vi "Serialize Proto.vi"(0 "protoFile ref in":u64, 3 "error in (no error)":errorcluster) -> (7 "protoFile ref out":u64, 8 "outBuffer":string, 10 "error out":errorcluster)   [LabVIEW 2019, in "gRPC Template Creation Utility.lvlib"]
uses:
  gRPC Template Creation Utility.lvlib
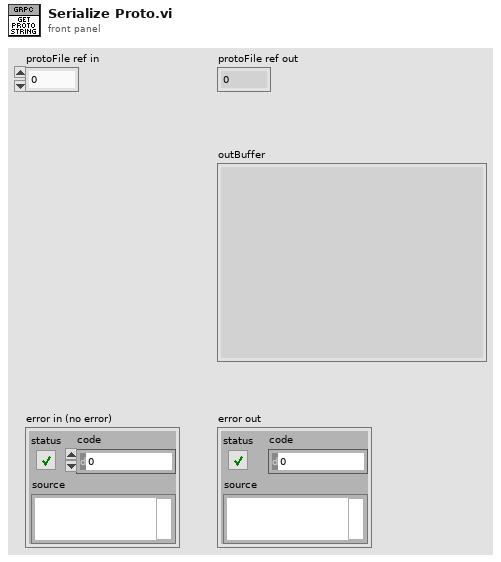
[diagram p1: front panel]
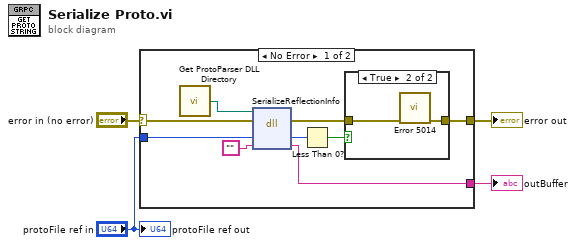
[diagram p0: block diagram]
diagram:
  n1 = case shown="No Error" "error in (no error)" {
    selector: "error in (no error)" -> [w13 w17]
    tunnel: [w11 w17] -> w3
    tunnel: "protoFile ref in" -> [w9 _]
    tunnel: [w5 _] -> w1
    frame No Error {
      n2 = call "Get ProtoParser DLL Directory.vi"() -> ("Proto Parser Directory"=w6:path)
      n3 = dll-call lib="C:/dev/grpc-labview-psn/build/Release/labview_grpc_generator.dll" fn="SerializeReflectionInfo"(path in=w6, error in=w13, "protoRef"=w9, "outBuffer"="") -> (error out=w12:errorcluster, "protoRef"=w8:u64, "outBuffer"=w5:string)  [unwired: 2 in, 1 out]
      n4 = Less Than 0?(x=w8) -> (x < 0?=w10:bool)
      n5 = case shown="True" w10 {
        tunnel: w12 -> [w14 w16]
        tunnel: [w14 w15] -> w11
        frame False {
        }
        frame True {
          n6 = call "Error 5014.vi"("error in (no error)"=w16) -> ("error out"=w15:errorcluster)  [unwired: 10 in]
        }
      }
    }
    frame Error {
    }
  }
  "error out" <- w3
  "outBuffer" <- w1
  "protoFile ref out" <- "protoFile ref in"
